vi "JUnit Basic.vi"() -> ()   [LabVIEW 2013]
doc: "This example illustrates the basic usage of <B>JUnit XML</B>."
uses:
  JUnit XML/Test Suite/Test Suite.lvclass
  JUnit XML/Test Case/Test Case.lvclass
panel:
  out "XML":string
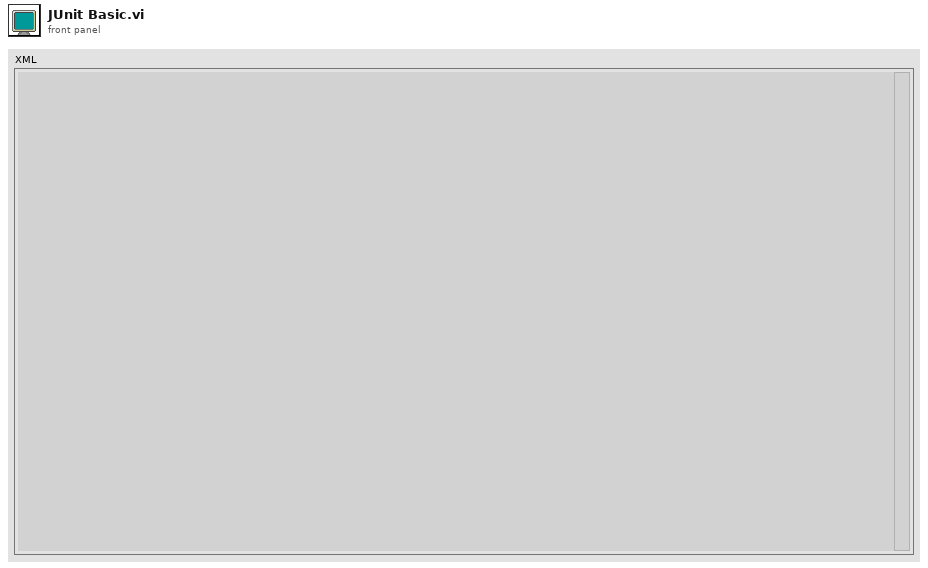
[diagram p1: front panel]
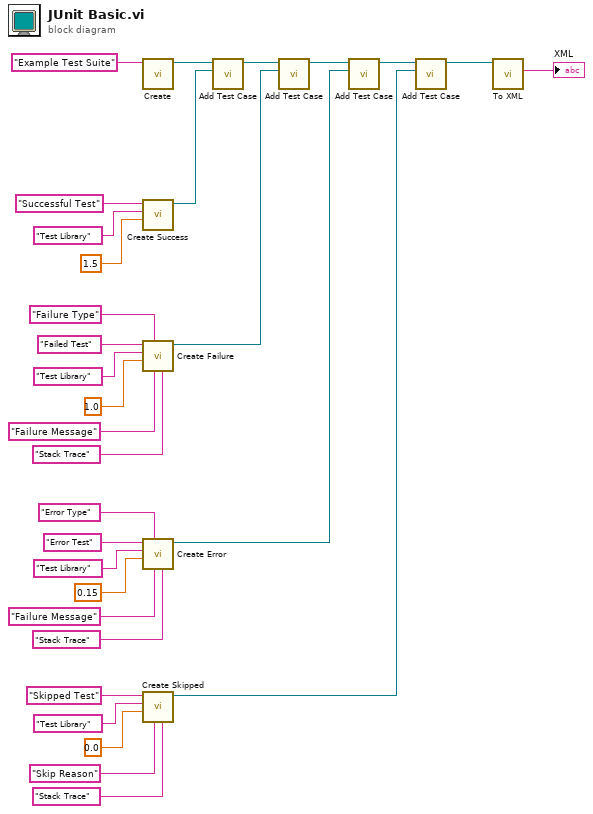
[diagram p0: block diagram]
diagram:
  n1 = call "Create.vi"("Name"="Example Test Suite") -> ("Test Suite"=w26:refnum<class "Test Suite.lvclass">)  [unwired: 9 in, 1 out]
  n2 = call "Create Success.vi"("Time"=1.5, "Classname"="Test Library", "Name"="Successful Test") -> ("Test Case"=w25:refnum<class "Test Case.lvclass">)  [unwired: 7 in, 1 out]
  n3 = call "Create Failure.vi"("Stack Trace"="Stack Trace", "Message"="Failure Message", "Type"="Failure Type", "Time"=1.0, "Classname"="Test Library", "Name"="Failed Test") -> ("Test Case"=w17:refnum<class "Test Case.lvclass">)  [unwired: 4 in, 1 out]
  n4 = call "Create Error.vi"("Stack Trace"="Stack Trace", "Message"="Failure Message", "Type"="Error Type", "Time"=0.15, "Classname"="Test Library", "Name"="Error Test") -> ("Test Case"=w9:refnum<class "Test Case.lvclass">)  [unwired: 4 in, 1 out]
  n5 = call "Create Skipped.vi"("Stack Trace"="Stack Trace", "Message"="Skip Reason", "Time"=0.0, "Classname"="Test Library", "Name"="Skipped Test") -> ("Test Case"=w1:refnum<class "Test Case.lvclass">)  [unwired: 5 in, 1 out]
  n6 = call "Add Test Case.vi"("Test Case"=w25, "Test Suite in"=w26) -> ("Test Suite out"=w18:refnum<class "Test Suite.lvclass">)  [unwired: 8 in, 1 out]
  n7 = call "Add Test Case.vi"("Test Case"=w17, "Test Suite in"=w18) -> ("Test Suite out"=w10:refnum<class "Test Suite.lvclass">)  [unwired: 8 in, 1 out]
  n8 = call "Add Test Case.vi"("Test Case"=w9, "Test Suite in"=w10) -> ("Test Suite out"=w3:refnum<class "Test Suite.lvclass">)  [unwired: 8 in, 1 out]
  n9 = call "Add Test Case.vi"("Test Case"=w1, "Test Suite in"=w3) -> ("Test Suite out"=w2:refnum<class "Test Suite.lvclass">)  [unwired: 8 in, 1 out]
  n10 = call-dynamic "To XML.vi"("Serializable in"=w2) -> ("XML"=→"XML":string)  [unwired: 9 in, 1 out]
